vi "Init.vi"(7 "VolatusAPI":refnum<class "VolatusAPI.lvclass">, 8 "error in (no error)":errorcluster, 11 "cRIO Power Status EStop in":refnum<class "cRIO Power Status EStop.lvclass">) -> (0 "error out":errorcluster, 3 "cRIO Power Status EStop out":refnum<class "cRIO Power Status EStop.lvclass">)   [LabVIEW 2025, in "VolatusControl.lvlib" / "cRIO Power Status EStop.lvclass"]
uses:
  cRIO Power Status EStop.lvclass
  cRIO Power Status EStop.lvclass/cRIO Power Status EStop.ctl
  Volatus/VolatusAPI/VolatusAPI.lvclass
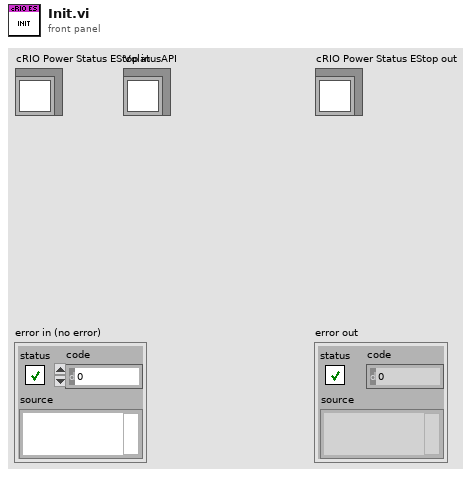
[diagram p1: front panel]
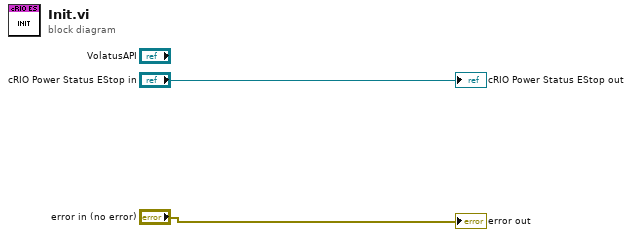
[diagram p0: block diagram]
diagram:
  "error out" <- "error in (no error)"
  "cRIO Power Status EStop out" <- "cRIO Power Status EStop in"
